vi "SA set All TDF OFF.vi"(8 "error in (no error)":errorcluster caption="에러 입력(에러 없음)", 11 "Instrument Manager 입력":refnum<class "Instrument Manager.lvclass">) -> (0 "error out":errorcluster caption="에러 출력", 3 "Instrument Manager 출력":refnum<class "Instrument Manager.lvclass">)   [LabVIEW 2023, in "Instrument Manager.lvclass"]
uses:
  Instrument Manager.lvclass
  Module/Spectrum Analyzer/Interface_Spectrum/Interface_Spectrum.lvclass
  62ba4117-f0ad-4209-9208-64b3993f5fb9.vi
  487f0394-b1ab-4e8d-9b7c-6458fb21627d.vi
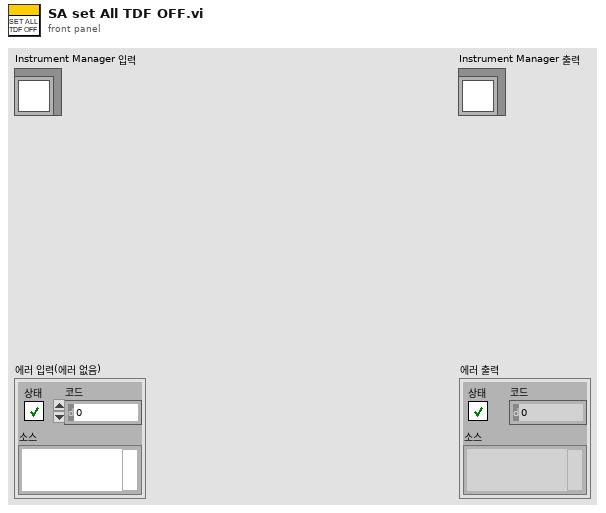
[diagram p1: front panel]
types:
  T1 = cluster{"Anritsu Call Box":refnum<class "Anritsu Call Box.lvclass">, "Spectrum Analyzer":refnum<class "Interface_Spectrum.lvclass">, "RF Switch Box":refnum<class "RF Filter Box.lvclass">, "Turn Table":refnum<class "Interface - Turn Table.lvclass">, "Mast":refnum<class "Interface - Mast.lvclass">, "3D Controller":refnum<class "Interface_3D Controller.lvclass">}
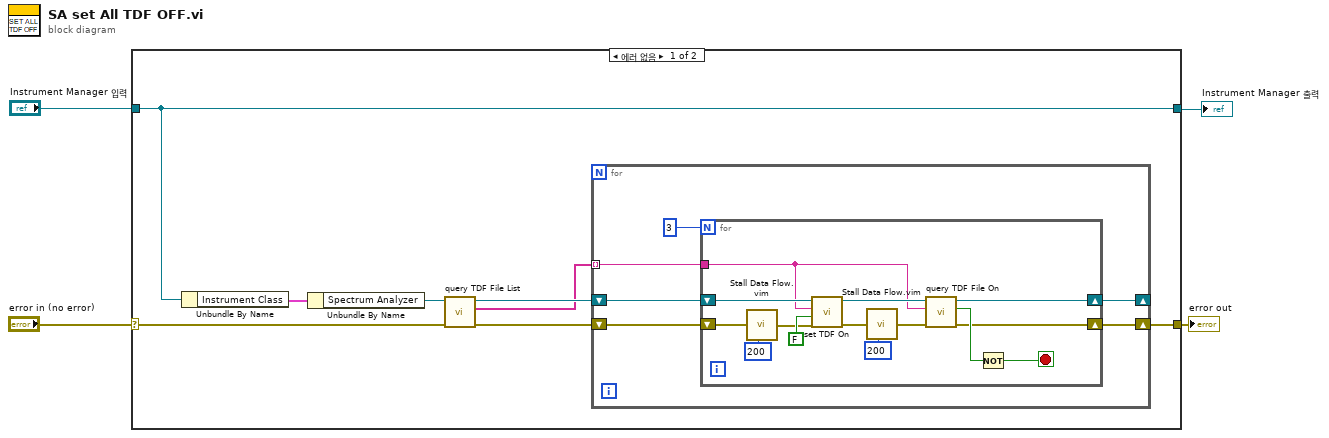
[diagram p0: block diagram]
diagram:
  n1 = case shown="에러 없음" "error in (no error)" {
    selector: "error in (no error)" -> [w12 w34]
    tunnel: [w5 w34] -> w3
    tunnel: [w11 w33] -> w1
    tunnel: "Instrument Manager 입력" -> [w11 w33]
    frame No Error {
      n2 = Unbundle By Name(w11) -> ("Instrument Class"=w10:T1)
      n3 = Unbundle By Name(w10) -> ("Spectrum Analyzer"=w9:refnum<class "Interface_Spectrum.lvclass">)
      n4 = call-dynamic "query TDF File List.vi"("error in (no error)"=w12, "Interface_Spectrum 입력"=w9) -> ("error out"=w8:errorcluster, "File List"=w6:string[], "Interface_Spectrum 출력"=w7:refnum<class "Interface_Spectrum.lvclass">)  [unwired: 7 in]
      n5 = for {
        shift-right: [w14] -> w5
        shift-left: w8 -> [w17]
        shift-right: [w13] -> _
        shift-left: w7 -> [w16]
        tunnel: w6 -> [w15] mode=indexing
        n6 = for {
          N: 3 -> [_]
          shift-right: [w26] -> w14
          shift-left: w17 -> [w20]
          shift-right: [w25] -> w13
          shift-left: w16 -> [w32]
          tunnel: w15 -> [w29]
          stop <- w27 stop-if-true
          n7 = call "Stall Data Flow.vim"("value in"=w20, "milliseconds to wait"=u32 200) -> ("value out"=w19:errorcluster)  [unwired: 1 out]
          n8 = call-dynamic "set TDF On.vi"("error in (no error)"=w19, "On?"=FALSE, "File Name"=w29, "Interface_Spectrum 입력"=w32) -> ("error out"=w24:errorcluster, "Interface_Spectrum 출력"=w31:refnum<class "Interface_Spectrum.lvclass">)  [unwired: 6 in]
          n9 = call "Stall Data Flow.vim"("value in"=w24, "milliseconds to wait"=u32 200) -> ("value out"=w23:errorcluster)  [unwired: 1 out]
          n10 = call-dynamic "query TDF File On.vi"("error in (no error)"=w23, "File Name"=w29, "Interface_Spectrum 입력"=w31) -> ("error out"=w26:errorcluster, "On?"=w28:bool, "Interface_Spectrum 출력"=w25:refnum<class "Interface_Spectrum.lvclass">)  [unwired: 6 in]
          n11 = Not(x=w28) -> (.not. x?=w27:bool)
        }
      }
    }
    frame Error {
    }
  }
  "error out" <- w3
  "Instrument Manager 출력" <- w1
